vi "DropVI_SimpleClient_Pub-Sub.vi"() -> ()   [LabVIEW 2013, in "MQTT Client.lvlib"]
uses:
  MQTT Client.lvlib
  Client class/Client.lvclass/Client.ctl
  <vilib>/LabVIEW Open Source Project/MQTT Connection/MQTT_Base/Base Class/MQTT_Base.lvclass/MQTT_Base.ctl
  <vilib>/LabVIEW Open Source Project/MQTT Control Packets/Control Packets/ControlPacket/QualityOfService -- enum.ctl
  <vilib>/LabVIEW Open Source Project/MQTT Control Packets/Control Packets/CONNECT/ConnectFlags -- cluster.ctl
  <vilib>/LabVIEW Open Source Project/MQTT Control Packets/Control Packets/PUBLISH/PUBLISH.lvclass
  Client class/Client.lvclass
  <vilib>/LabVIEW Open Source Project/MQTT Connection/MQTT_Base/Base Class/MQTT_Base.lvclass
  <vilib>/LabVIEW Open Source Project/MQTT Control Packets/Control Packets/CONNECT/CONNECT.lvclass
  <vilib>/LabVIEW Open Source Project/MQTT Control Packets/Control Packets/ControlPacket/ControlPacket.lvclass
  <vilib>/LabVIEW Open Source Project/Connection/Connection/Connection.lvclass
  <vilib>/LabVIEW Open Source Project/Connection/Connection.TCP/Connection.TCP.lvclass
  <vilib>/LabVIEW Open Source Project/Connection/Connection.LocalQueue/Connection.LocalQueue.lvclass
panel:
  out "Published":bool
  out "last error":errorcluster
  out "Unsuback":bool
  in  "Subscribe":bool
  in  "Connection":bool
  out "Waveform Chart":dbl(graph)
  out "Suback":bool
  in  "Stop Client":bool
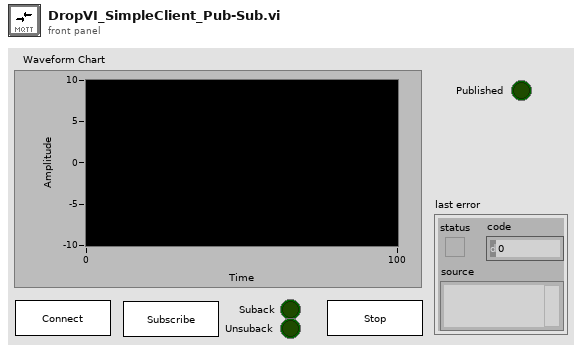
[diagram p1: front panel]
types:
  T1 = typedef "MQTT Client.lvlib/Client.lvclass/Public Events -- cluster.ctl" = cluster{"Connection Status":refnum<user-event>, "Connected":refnum<user-event>, "Application Message":refnum<user-event>}
  T2 = typedef "MQTT Base.lvlib/MQTT_Base.lvclass/Public Events -- cluster.ctl" = cluster{"Stop Event":refnum<user-event>, "Error Event":refnum<user-event>, "Inbound Message":refnum<user-event>}
  T3 = typedef "MQTT_Control_Packets.lvlib/ControlPacket.lvclass/QualityOfService -- enum.ctl" = enum16{"0 (At Most Once)", "1 (At Least Once)", "2 (Exactly Once)"}
  T4 = typedef "MQTT_Control_Packets.lvlib/CONNECT.lvclass/ConnectFlags -- cluster.ctl" = cluster{"Reserved":bool, "Clean Session":bool, "Will Flag":bool, "Will QoS 1":bool, "Will QoS 2":bool, "Will Retain":bool, "Password Flag":bool, "User Name Flag":bool}
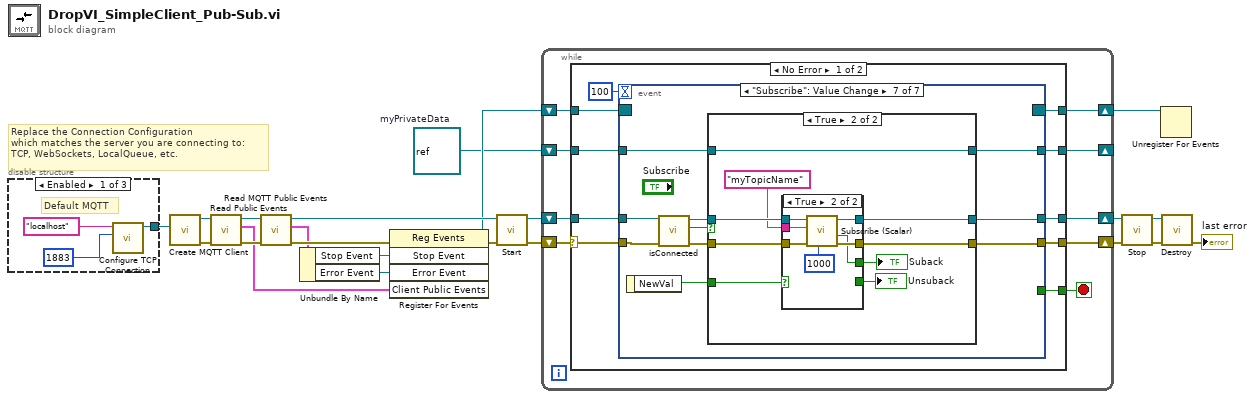
[diagram p0: block diagram]
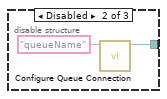
[diagram p2: hidden frame]
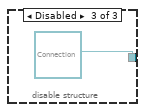
[diagram p3: hidden frame]
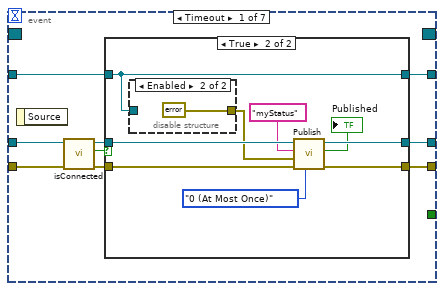
[diagram p4: hidden frame]
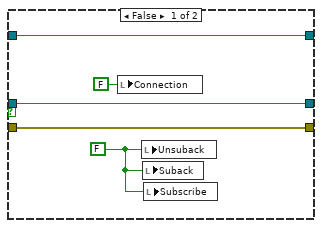
[diagram p5: hidden frame]
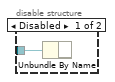
[diagram p6: hidden frame]
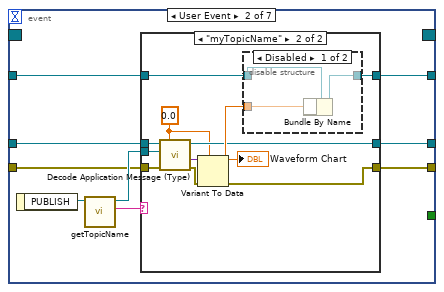
[diagram p7: hidden frame]
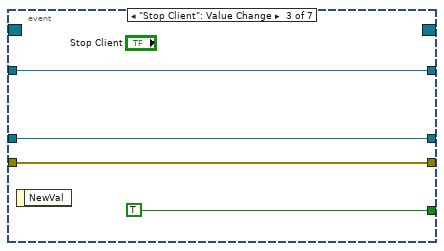
[diagram p10: hidden frame]
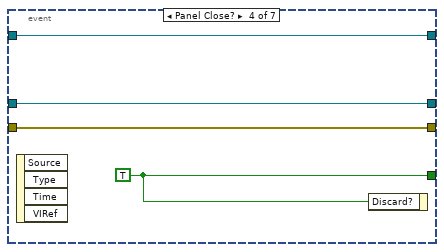
[diagram p11: hidden frame]
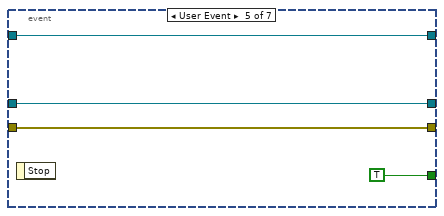
[diagram p12: hidden frame]
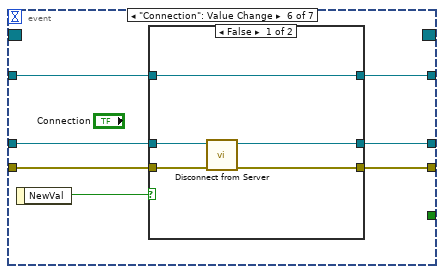
[diagram p13: hidden frame]
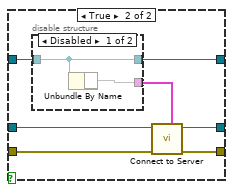
[diagram p14: hidden frame]
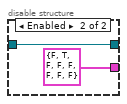
[diagram p15: hidden frame]
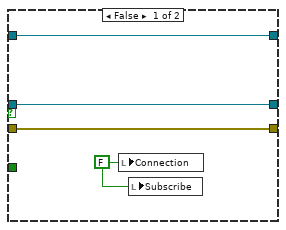
[diagram p16: hidden frame]
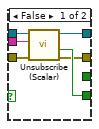
[diagram p17: hidden frame]
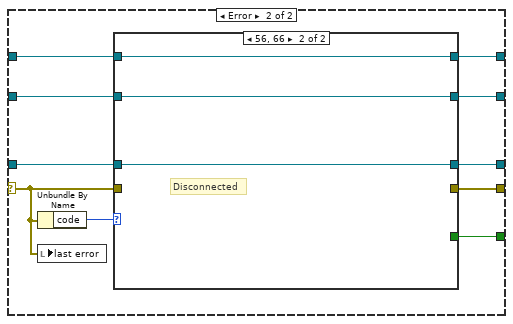
[diagram p18: hidden frame]
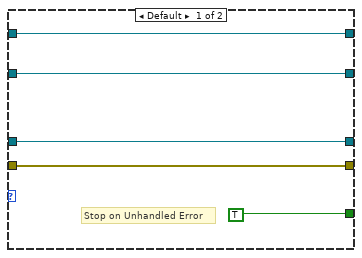
[diagram p19: hidden frame]
diagram:
  w2 = refnum<class> refnum  # myPrivateData
  # "Replace the Connection Configuration\nwhich matches the server you are connecting to:\nTCP, WebSockets, LocalQueue, etc."
  n1 = disable-structure shown="Enabled" {
    disable-tunnel: [w23 w27 refnum<class "Connection.lvclass"> refnum ("Connection Configuration")] -> w1
    frame Enabled {
      # "Default MQTT"
      n2 = call <vilib>:"Configure TCP Connection.vi"("remote port (80)"=u16 1883, "address (localhost)"="localhost") -> ("Connection.TCP"=w23:refnum<class "Connection.TCP.lvclass">)  [unwired: 8 in, 1 out]
    }
    frame Disabled {
      n3 = call <vilib>:"Configure Queue Connection.vi"("Queue Name"="queueName") -> ("Connection.LocalQueue"=w27:refnum<class "Connection.LocalQueue.lvclass">)  [unwired: 9 in, 1 out]
    }
    frame Disabled {
    }
  }
  n4 = call "Create MQTT Client.vi"("Connection Configuration"=w1) -> ("error out"=w20:errorcluster, "Client out"=w22:refnum<class "Client.lvclass">)  [unwired: 9 in]
  n5 = call "Read Public Events.vi"("error in (no error)"=w20, "Client in"=w22) -> ("error out"=w19:errorcluster, "Client Public Events"=w17:T1, "Client out"=w21:refnum<class "Client.lvclass">)  [unwired: 7 in]
  n6 = call <vilib>:"Read MQTT Public Events.vi"("error in (no error)"=w19, "MQTT_Base in"=w21) -> ("error out"=w18:errorcluster, "MQTT Public Events"=w10:T2, "MQTT_Base out"=w15:refnum<class "Client.lvclass">)  [unwired: 7 in]
  n7 = Unbundle By Name(w10) -> ("Stop Event"=w12:refnum<user-event>, "Error Event"=w11:refnum<user-event>)
  n8 = register-events(error in=w18, w12, w11, w17) -> (reference out=w14:refnum<event-registration>, error out=w16:errorcluster)  [unwired: 1 in]
  n9 = call <vilib>:"Start.vi"("error in (no error)"=w16, "MQTT_Base in"=w15) -> ("error out"=w4:errorcluster, "MQTT_Base out"=w5:refnum<class "Client.lvclass">)  [unwired: 7 in, 1 out]
  n10 = while {
    shift-right: [w36] -> w13
    shift-left: w14 -> [w37]
    shift-right: [w33] -> w8
    shift-left: w5 -> [w34]
    shift-right: [w35] -> w6
    shift-left: w4 -> [w31]
    shift-right: [w29] -> _
    shift-left: w2 -> [w30]
    stop <- w32 stop-if-true
    n11 = case shown="No Error" w31 {
      selector: w31 -> [w40 w174]
      tunnel: w37 -> [w47 w173]
      tunnel: [w46 w172] -> w36
      tunnel: [w45 w177] -> w35
      tunnel: w34 -> [w43 w178]
      tunnel: [w42 w180] -> w33
      tunnel: [w41 w176] -> w32
      tunnel: w30 -> [w39 w175]
      tunnel: [w38 w171] -> w29
      frame No Error {
        n12 = event shown="[6] \"Subscribe\": Value Change" {
          selector: w47 -> [_ _ _ _ _ _ _]
          dyn-events: [_ _ _ _ _ _ _] -> w46
          timeout: 100 -> [_ _ _ _ _ _ _]
          tunnel: w40 -> [w52 w78 w102 w105 w111 w114 w142]
          tunnel: [w55 w75 w102 w105 w111 w115 w143] -> w45
          tunnel: [_ _ TRUE w107 TRUE _ _] -> w41
          tunnel: w43 -> [w54 w79 w103 w106 w109 w118 w141]
          tunnel: [w56 w77 w103 w106 w109 w116 w144] -> w42
          tunnel: w39 -> [w49 w74 w100 w104 w108 w112 w136]
          tunnel: [w48 w73 w100 w104 w108 w113 w135] -> w38
          event Timeout {
            n13 = event-data() -> ()  [unwired: 1 in, 1 out]
            n14 = call "isConnected.vi"("error in (no error)"=w52, "Client in"=w54) -> ("error out"=w51:errorcluster, "connected"=w50:bool, "Client out"=w53:refnum<class "Client.lvclass">)  [unwired: 7 in]
            n15 = case shown="True" w50 {
              tunnel: [w61 w69] -> w56
              tunnel: [w60 w67] -> w55
              tunnel: w53 -> [w61 w70]
              tunnel: w51 -> [w60 w68]
              tunnel: w49 -> [w57 w65]
              tunnel: [w57 w65] -> w48
              frame False {
                w59 = FALSE
                n16 = local write "Connection"(FALSE ("Connection")) -> ()
                n17 = local write "Unsuback"(w59) -> ()
                n18 = local write "Suback"(w59) -> ()
                n19 = local write "Subscribe"(w59) -> ()
              }
              frame True {
                n20 = disable-structure shown="Enabled" {
                  disable-tunnel: w65 -> [w71 _]
                  disable-tunnel: [_ errorcluster {"status"=FALSE, "code"=0, "source"=""} ("error constant")] -> w64
                  frame Disabled {
                    n21 = Unbundle By Name(w71) -> ()  [unwired: 1 out]
                  }
                  frame Enabled {
                  }
                }
                n22 = call "Publish.vi"("QoS"=QualityOfService_--_enum."0 (At Most Once)", "error in (no error)"=w68, "Payload"=w64, "Topic Name (empty: Payload name)"="myStatus", "Client in"=w70) -> ("error out"=w67:errorcluster, "Published"=→"Published":bool, "Client out"=w69:refnum<class "Client.lvclass">)  [unwired: 4 in]
              }
            }
          }
          event User Event {
            n23 = event-data() -> ("PUBLISH"=w81:refnum<class "PUBLISH.lvclass">)  [unwired: 1 in]
            n24 = call <vilib>:"getTopicName.vi"("PUBLISH in"=w81) -> ("Topic"=w76:string, "PUBLISH out"=w80:refnum<class "PUBLISH.lvclass">)  [unwired: 8 in, 1 out]
            n25 = case shown="\"myTopicName\"" w76 {
              tunnel: w80 -> [_ w90]
              tunnel: w79 -> [w84 w91]
              tunnel: w78 -> [w83 w89]
              tunnel: [w84 w86] -> w77
              tunnel: [w83 w95] -> w75
              tunnel: w74 -> [w82 w94]
              tunnel: [w82 w93] -> w73
              frame Default {
              }
              frame "myTopicName" {
                w85 = 0.0
                n26 = call "Decode Application Message (Type).vi"("Type"=w85, "error in (no error)"=w89, "PUBLISH"=w90, "Client in"=w91) -> ("error out"=w88:errorcluster, "Payload"=w87:variant, "Client out"=w86:refnum<class "Client.lvclass">)  [unwired: 4 in, 1 out]
                n27 = Variant To Data(error in=w88, type=w85, Variant=w87) -> (data=w92:dbl, error out=w95:errorcluster)
                "Waveform Chart" <- w92
                n28 = disable-structure shown="Disabled" {
                  disable-tunnel: w94 -> [w96 w99]
                  disable-tunnel: [w98 w99] -> w93
                  disable-tunnel: w92 -> [w97 _]
                  frame Disabled {
                    n29 = Bundle By Name(cluster=w96, w97) -> (w98:refnum<class>)
                  }
                  frame Enabled {
                  }
                }
              }
            }
          }
          event "Stop Client": Value Change {
            n30 = event-data() -> ()  [unwired: 1 in, 1 out]
          }
          event Panel Close? {
            w107 = TRUE
            n31 = event-data() -> ()  [unwired: 1 in, 4 out]
            n32 = event-data("Discard?"=w107) -> ()  [unwired: 1 in, 1 out]
          }
          event User Event {
            n33 = event-data() -> ()  [unwired: 1 in, 1 out]
          }
          event "Connection": Value Change {
            n34 = event-data() -> ("NewVal"=w117:bool)  [unwired: 1 in]
            n35 = case shown="False" w117 {
              tunnel: w118 -> [w123 w130]
              tunnel: [w122 w127] -> w116
              tunnel: [w121 w128] -> w115
              tunnel: w114 -> [w120 w129]
              tunnel: [w119 w125] -> w113
              tunnel: w112 -> [w119 w126]
              frame False {
                n36 = call "Disconnect from Server.vi"("error in (no error)"=w120, "Client in"=w123) -> ("error out"=w121:errorcluster, "Client out"=w122:refnum<class "Client.lvclass">)  [unwired: 7 in, 1 out]
              }
              frame True {
                n37 = disable-structure shown="Disabled" {
                  disable-tunnel: w126 -> [w132 w134]
                  disable-tunnel: [w132 w134] -> w125
                  disable-tunnel: [w131 T4 {"Reserved"=FALSE, "Clean Session"=TRUE, "Will Flag"=FALSE, "Will QoS 1"=FALSE, "Will QoS 2"=FALSE, "Will Retain"=FALSE, "Password Flag"=FALSE, "User Name Flag"=FALSE} ("Connect Flags")] -> w124
                  frame Disabled {
                    n38 = Unbundle By Name(w132) -> (w131)
                  }
                  frame Enabled {
                  }
                }
                n39 = call "Connect to Server.vi"("Connect Flags"=w124, "error in (no error)"=w129, "Client in"=w130) -> ("error out"=w128:errorcluster, "Client out"=w127:refnum<class "Client.lvclass">)  [unwired: 5 in, 2 out]
              }
            }
          }
          event "Subscribe": Value Change {
            n40 = event-data() -> ("NewVal"=w137:bool)  [unwired: 1 in]
            n41 = call "isConnected.vi"("error in (no error)"=w142, "Client in"=w141) -> ("error out"=w139:errorcluster, "connected"=w138:bool, "Client out"=w140:refnum<class "Client.lvclass">)  [unwired: 7 in]
            n42 = case shown="True" w138 {
              tunnel: [w148 w157] -> w144
              tunnel: [w147 w156] -> w143
              tunnel: w140 -> [w148 w155]
              tunnel: w139 -> [w147 w154]
              tunnel: w137 -> [_ w152]
              tunnel: w136 -> [w145 w149]
              tunnel: [w145 w149] -> w135
              frame False {
                w146 = FALSE ("Connection")
                n43 = local write "Connection"(w146) -> ()
                n44 = local write "Subscribe"(w146) -> ()
              }
              frame True {
                n45 = case shown="True" w152 {
                  tunnel: [w160 w169] -> w157
                  tunnel: [w158 w166] -> w156
                  tunnel: w155 -> [w163 w170]
                  tunnel: w154 -> [w162 w167]
                  tunnel: "myTopicName" ("Topic Name (empty: Payload name)") -> [w161 w168]
                  tunnel: [_ w165] -> w151
                  tunnel: [w159 _] -> w150
                  frame False {
                    n46 = call "Unsubscribe (Scalar).vi"("error in (no error)"=w162, "Topic Filter"=w161, "Client in"=w163) -> ("error out"=w158:errorcluster, "Ack"=w159:bool, "Client out"=w160:refnum<class "Client.lvclass">)  [unwired: 6 in]
                  }
                  frame True {
                    n47 = call "Subscribe (Scalar).vi"("timeout (1000ms)"=1000 ("timeout (100ms)"), "error in (no error)"=w167, "Topic Filter"=w168, "Client in"=w170) -> ("error out"=w166:errorcluster, "Ack"=w165:bool, "Client out"=w169:refnum<class "Client.lvclass">)  [unwired: 5 in]
                  }
                }
                "Unsuback" <- w150
                "Suback" <- w151
              }
            }
          }
        }
      }
      frame Error {
        n48 = Unbundle By Name(w174) -> ("code"=w179:i32)
        n49 = local write "last error"(w174) -> ()
        n50 = case shown="56, 66" w179 {
          tunnel: w178 -> [w185 w188]
          tunnel: [w185 w188] -> w180
          tunnel: w174 -> [w184 _]
          tunnel: [w184 _] -> w177
          tunnel: [TRUE _] -> w176
          tunnel: w175 -> [w181 w186]
          tunnel: w173 -> [w182 w187]
          tunnel: [w182 w187] -> w172
          tunnel: [w181 w186] -> w171
          frame Default {
            # "Stop on Unhandled Error"
          }
          frame 56, 66 {
            # "Disconnected"
          }
        }
      }
    }
  }
  n51 = call <vilib>:"Stop.vi"("error in (no error)"=w6, "MQTT_Base in"=w8) -> ("error out"=w7:errorcluster, "MQTT_Base out"=w9:refnum<class "Client.lvclass">)  [unwired: 7 in, 1 out]
  n52 = Unregister For Events(event registration refnum=w13) -> ()  [unwired: 1 in, 1 out]
  n53 = call <vilib>:"Destroy.vi"("error in (no error)"=w7, "MQTT_Base in"=w9) -> ("error out"=→"last error":errorcluster)  [unwired: 8 in, 1 out]
